vi "New Message.vi"(0 "Message Maker in":refnum<class "Message Maker.lvclass">, 5 "Method Qualified Name":string, 11 "error in (no error)":errorcluster, 12 "Message Type":T1) -> (3 "Message Recipient Type":T2, 4 "Message Maker out":refnum<class "Message Maker.lvclass">, 6 "References":T3, 8 "AF Library FQN":string, 10 "Async AF Library FQN":string, 14 "Updating?":bool, 15 "error out":errorcluster)   [LabVIEW 2023, in "Message Maker.lvclass"]
doc: "Sets up the method to be built. If this is a new message, it will copy over the template. If this is a message to be updated it resets the old message\n\nAuthor: Derek Trepanier\nCopyright: MGI 2015"
uses:
  Message Maker.lvclass
  Scripting Refs.ctl
  Message Recipient Type.ctl
  Message Type.ctl
  Message Maker.lvclass/Message Maker.ctl
  <vilib>/Utility/error.llb/Error Cluster From Error Code.vi
  <vilib>/ErrorRing/Error Ring.xnode
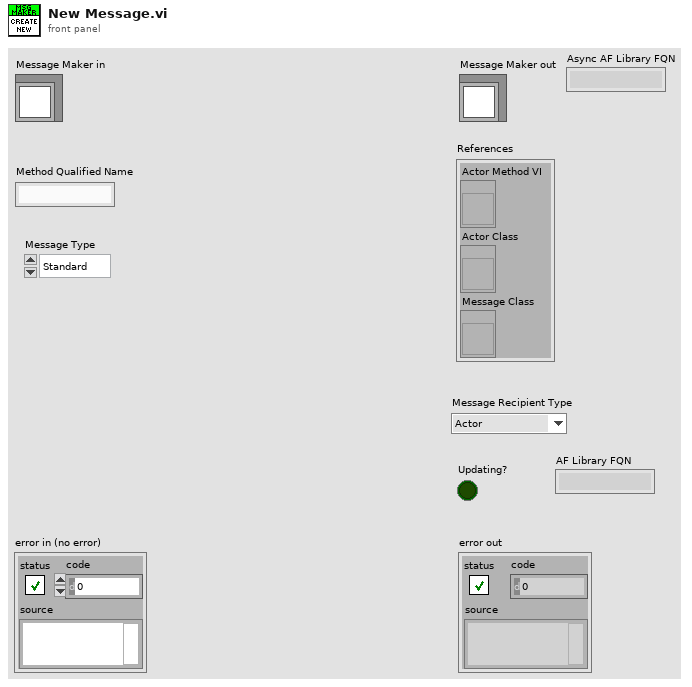
[diagram p1: front panel]
types:
  T1 = typedef "Message Maker.lvclass/Message Type.ctl" = enum16{"Standard", "Async"}
  T2 = typedef "Message Maker.lvclass/Message Recipient Type.ctl" = enum16{"Actor", "Interface", "Async Actor"}
  T3 = typedef "Message Maker.lvclass/Scripting Refs.ctl" = cluster{"Actor Method VI":refnum<vi>, "Actor Class":refnum<vi>, "Message Class":refnum<vi>}
  T4 = typedef "Message Maker.lvclass/Messages Map.ctl" = map{string, T5}
  T5 = typedef "Message Maker.lvclass/Message Details.ctl" = cluster{"Message Ref":refnum<vi>, "Message Type":T1}
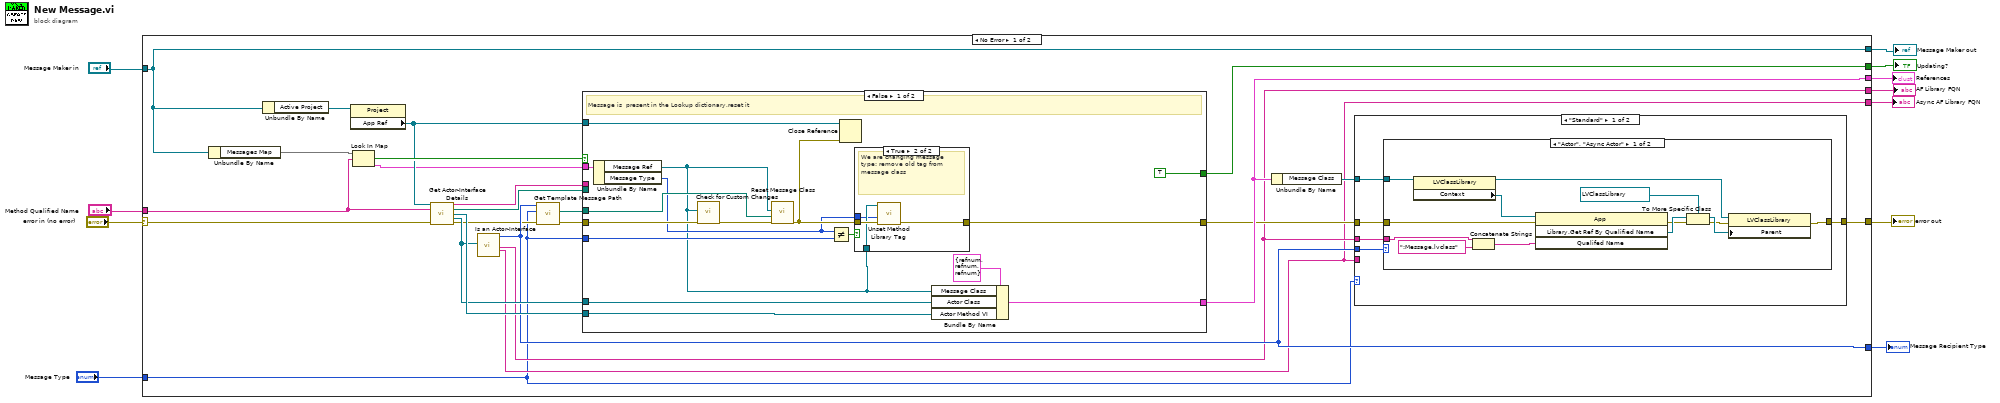
[diagram p0: block diagram]
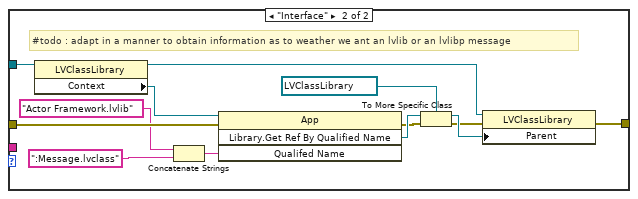
[diagram p2: hidden frame]
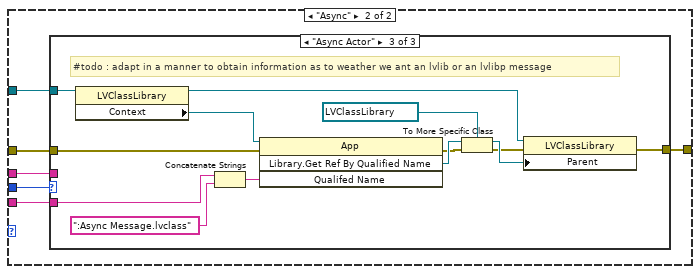
[diagram p3: hidden frame]
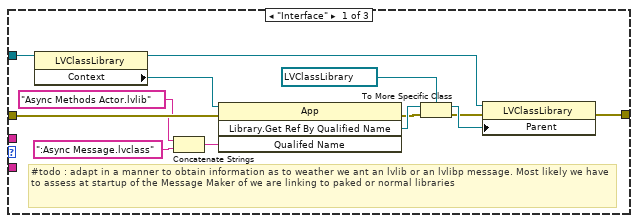
[diagram p4: hidden frame]
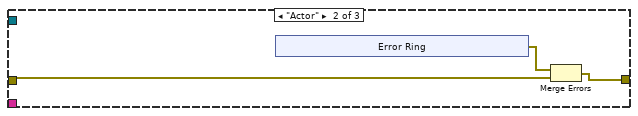
[diagram p5: hidden frame]
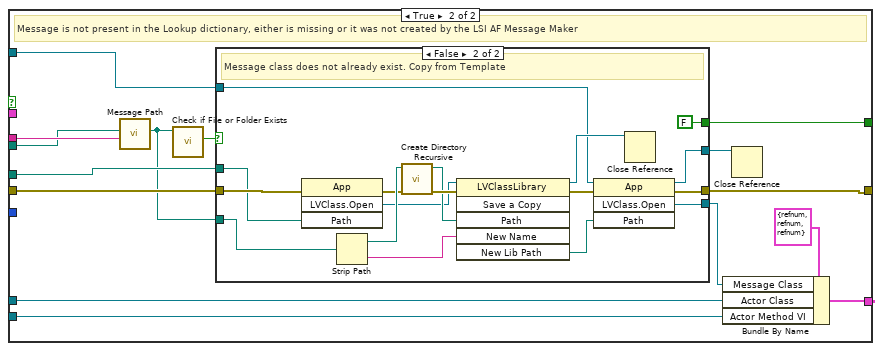
[diagram p7: hidden frame]
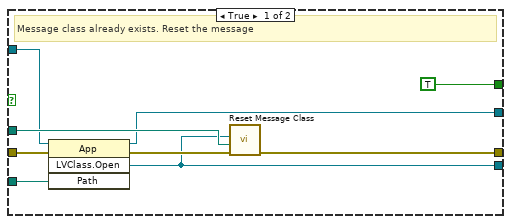
[diagram p8: hidden frame]
diagram:
  n1 = case shown="No Error" "error in (no error)" {
    selector: "error in (no error)" -> [w28 w169]
    tunnel: [w31 w169] -> w10
    tunnel: [w20 w168] -> w8
    tunnel: "Message Maker in" -> [w20 w168]
    tunnel: "Method Qualified Name" -> [w27 _]
    tunnel: [w33 _] -> w6
    tunnel: [w34 _] -> w5
    tunnel: [w15 _] -> w4
    tunnel: [w18 _] -> w3
    tunnel: "Message Type" -> [w12 _]
    tunnel: [w14 _] -> w1
    frame No Error {
      n2 = Unbundle By Name(w20) -> ("Messages Map"=w19:T4)
      n3 = Unbundle By Name(w20) -> ("Active Project"=w29:refnum<vi>)
      n4 = property class="Project"(reference=w29) -> ("App Ref"=w26:refnum<vi>)  [unwired: 1 in, 2 out]
      n5 = Look In Map(map=w19, key=w27) -> (key not found?=w35:bool, value=w13:T5)  [unwired: 1 in]
      n6 = call "Get Actor-Interface Details.vi"("Application"=w26, "Method Qualified Name"=w27, "error in (no error)"=w28) -> ("Actor Name"=w25:string, "Actor Path"=w24:path, "Actor Method VI Reference"=w23:refnum<vi>, "Actor Reference"=w21:refnum<vi>, "error out"=w17:errorcluster)  [unwired: 8 in]
      n7 = call "Is an Actor-Interface.vi"("Class in"=w21) -> ("Message Recipient Type"=w18:T2, "AF Library FQN"=w15:string, "Async AF Library FQN"=w14:string)  [unwired: 14 in, 2 out]
      n8 = call "Get Template Message Path.vi"("error in"=w17, "Message Type"=w12, "Message Recipient Type"=w18) -> ("error out"=w16:errorcluster, "appended path"=w22:path)  [unwired: 7 in]
      n9 = case shown="False" w35 {
        tunnel: [w119 w128] -> w33
        tunnel: w16 -> [w117 w139]
        tunnel: [w112 w129] -> w30
        tunnel: w22 -> [w121 w137]
        tunnel: [TRUE w136] -> w34
        tunnel: w26 -> [w115 w135]
        tunnel: w25 -> [_ w134]
        tunnel: w24 -> [_ w133]
        tunnel: w21 -> [w111 w132]
        tunnel: w23 -> [w114 w131]
        tunnel: w13 -> [w110 _]
        tunnel: w12 -> [w109 _]
        frame False {
          # "Message is  present in the Lookup dictionary,reset it"
          n10 = Unbundle By Name(w110) -> ("Message Ref"=w106:refnum<vi>, "Message Type"=w107:T1)
          n11 = call "Check for Custom Changes.vi"("error in (no error)"=w117, "Message Class"=w106) -> ("error out"=w116:errorcluster)  [unwired: 9 in]
          n12 = call "Reset Message Class.vi"("error in (no error)"=w116, "Template Path"=w121, "Message Class"=w106) -> ("error out"=w113:errorcluster)  [unwired: 8 in]
          n13 = Not Equal?(x=w107, y=w109) -> (x != y?=w108:bool)
          n14 = Close Reference(reference=w115, error in (no error)=w113) -> ()  [unwired: 1 out]
          n15 = case shown="True" w108 {
            tunnel: w113 -> [w122 w126]
            tunnel: [w122 w125] -> w112
            tunnel: w106 -> [_ w124]
            tunnel: w107 -> [_ w123]
            frame False {
            }
            frame True {
              # "We are changing message type: remove old tag from message class"
              n16 = call "Unset Method Library Tag.vi"("error in (no error)"=w126, "Message Type"=w123, "LVClassLibrary in"=w124) -> ("error out"=w125:errorcluster)  [unwired: 7 in, 1 out]
            }
          }
          n17 = Bundle By Name(cluster=T3 {"Actor Method VI"=refnum, "Actor Class"=refnum, "Message Class"=refnum} ("References"), "Message Class"=w106, "Actor Class"=w111, "Actor Method VI"=w114) -> (w119:T3)
        }
        frame True {
          # "Message is not present in the Lookup dictionary, either is missing or it was not created by the LSI AF Message Maker"
          n18 = call "Message Path.vi"("Message Method"=w134, "Class Path"=w133) -> ("Message Class Path"=w130:path)  [unwired: 9 in]
          n19 = call <vilib>:"Check if File or Folder Exists.vi"("path"=w130) -> ("file or folder exists?"=w127:bool)  [unwired: 8 in, 2 out]
          n20 = case shown="False" w127 {
            tunnel: w130 -> [w148 w161]
            tunnel: w139 -> [w145 w159]
            tunnel: w135 -> [w149 w158]
            tunnel: [w143 w155] -> w140
            tunnel: [w144 w154] -> w129
            tunnel: [w147 w153] -> w138
            tunnel: w137 -> [w150 w152]
            tunnel: [TRUE FALSE] -> w136
            frame True {
              # "Message class already exists. Reset the message"
              n21 = invoke class="App" method="LVClass.Open"(reference=w149, error in=w145, "Path"=w148) -> (reference out=w147:refnum<vi>, error out=w146:errorcluster, "LVClass.Open"=w143:refnum<vi>)  [unwired: 1 in, 1 out]
              n22 = call "Reset Message Class.vi"("error in (no error)"=w146, "Template Path"=w150, "Message Class"=w143) -> ("error out"=w144:errorcluster)  [unwired: 8 in]
            }
            frame False {
              # "Message class does not already exist. Copy from Template"
              n23 = invoke class="App" method="LVClass.Open"(error in=w159, "Path"=w152) -> (error out=w160:errorcluster, "LVClass.Open"=w163:refnum<vi>)  [unwired: 2 in, 2 out]
              n24 = Strip Path(path=w161) -> (stripped path=w165:path, name=w162:string)
              n25 = call <vilib>:"Create Directory Recursive.vi"("error in (no error)"=w160, "directory"=w165) -> ("error out"=w167:errorcluster, "directory copy"=w166:path)  [unwired: 3 in, 1 out]
              n26 = invoke class="LVClassLibrary" method="Save a Copy"(reference=w163, error in=w167, "Path"=w166, "New Name"=w162) -> (reference out=w164:refnum<vi>, error out=w156:errorcluster, "New Lib Path"=w157:path)  [unwired: 2 in, 3 out]
              n27 = invoke class="App" method="LVClass.Open"(reference=w158, error in=w156, "Path"=w157) -> (reference out=w153:refnum<vi>, error out=w154:errorcluster, "LVClass.Open"=w155:refnum<vi>)  [unwired: 1 in, 1 out]
              n28 = Close Reference(reference=w164) -> ()  [unwired: 1 in, 1 out]
            }
          }
          n29 = Bundle By Name(cluster=T3 {"Actor Method VI"=refnum, "Actor Class"=refnum, "Message Class"=refnum} ("References"), "Message Class"=w140, "Actor Class"=w132, "Actor Method VI"=w131) -> (w128:T3)
          n30 = Close Reference(reference=w138) -> ()  [unwired: 1 in, 1 out]
        }
      }
      n31 = Unbundle By Name(w33) -> ("Message Class"=w32:refnum<vi>)
      n32 = case shown="\"Standard\"" w12 {
        tunnel: w32 -> [w40 w72]
        tunnel: [w39 w71] -> w31
        tunnel: w30 -> [w38 w70]
        tunnel: w15 -> [w37 w69]
        tunnel: w18 -> [w36 w68]
        tunnel: w14 -> [_ w67]
        frame "Standard" {
          n33 = case shown="\"Actor\", \"Async Actor\"" w36 {
            tunnel: w40 -> [w53 w66]
            tunnel: [w52 w65] -> w39
            tunnel: w38 -> [w51 w64]
            tunnel: w37 -> [w41 _]
            frame "Actor", "Async Actor" {
              n34 = property class="LVClassLibrary"(reference=w53) -> (reference out=w50:refnum<vi>, "Context"=w49:refnum<vi>)  [unwired: 1 in, 1 out]
              n35 = Concatenate Strings(w41, ":Message.lvclass" ("string")) -> (w42:string)
              n36 = invoke class="App" method="Library.Get Ref By Qualified Name"(reference=w49, error in=w51, "Qualifed Name"=w42) -> (error out=w45:errorcluster, "Library.Get Ref By Qualified Name"=w48:refnum<vi>)  [unwired: 1 in, 2 out]
              n37 = To More Specific Class(target class=refnum<vi> refnum ("Parent Class"), reference=w48, error in=w45) -> (specific class reference=w46:refnum<vi>, error out=w44:errorcluster)
              n38 = property class="LVClassLibrary"(reference=w50, error in=w44, "Parent"=w46) -> (error out=w52:errorcluster)  [unwired: 1 out]
            }
            frame "Interface" {
              # "#todo : adapt in a manner to obtain information as to weather we ant an lvlib or an lvlibp message"
              n39 = property class="LVClassLibrary"(reference=w66) -> (reference out=w63:refnum<vi>, "Context"=w62:refnum<vi>)  [unwired: 1 in, 1 out]
              n40 = Concatenate Strings("Actor Framework.lvlib" ("Actor Class"), ":Message.lvclass" ("string")) -> (w55:string)
              n41 = invoke class="App" method="Library.Get Ref By Qualified Name"(reference=w62, error in=w64, "Qualifed Name"=w55) -> (error out=w58:errorcluster, "Library.Get Ref By Qualified Name"=w61:refnum<vi>)  [unwired: 1 in, 2 out]
              n42 = To More Specific Class(target class=refnum<vi> refnum ("Parent Class"), reference=w61, error in=w58) -> (specific class reference=w59:refnum<vi>, error out=w57:errorcluster)
              n43 = property class="LVClassLibrary"(reference=w63, error in=w57, "Parent"=w59) -> (error out=w65:errorcluster)  [unwired: 1 out]
            }
          }
        }
        frame "Async" {
          n44 = case shown="\"Async Actor\"" w68 {
            tunnel: w72 -> [w85 _ w105]
            tunnel: [w84 w86 w104] -> w71
            tunnel: w70 -> [w83 w87 w103]
            tunnel: w69 -> [_ _ _]
            tunnel: w67 -> [_ _ w93]
            frame "Interface" {
              # "#todo : adapt in a manner to obtain information as to weather we ant an lvlib or an lvlibp message. Most likely we have to assess at startup of the Message Maker of we are linking to paked or normal libraries"
              n45 = property class="LVClassLibrary"(reference=w85) -> (reference out=w82:refnum<vi>, "Context"=w81:refnum<vi>)  [unwired: 1 in, 1 out]
              n46 = Concatenate Strings("Async Methods Actor.lvlib" ("Actor Class"), ":Async Message.lvclass" ("string")) -> (w74:string)
              n47 = invoke class="App" method="Library.Get Ref By Qualified Name"(reference=w81, error in=w83, "Qualifed Name"=w74) -> (error out=w77:errorcluster, "Library.Get Ref By Qualified Name"=w80:refnum<vi>)  [unwired: 1 in, 2 out]
              n48 = To More Specific Class(target class=refnum<vi> refnum ("Parent Class"), reference=w80, error in=w77) -> (specific class reference=w78:refnum<vi>, error out=w76:errorcluster)
              n49 = property class="LVClassLibrary"(reference=w82, error in=w76, "Parent"=w78) -> (error out=w84:errorcluster)  [unwired: 1 out]
            }
            frame "Actor" {
              n50 = xnode "Error Ring"() -> ("error out"=w88:errorcluster)
              n51 = Merge Errors(w88, w87) -> (w86:errorcluster)
            }
            frame "Async Actor" {
              # "#todo : adapt in a manner to obtain information as to weather we ant an lvlib or an lvlibp message"
              n52 = property class="LVClassLibrary"(reference=w105) -> (reference out=w102:refnum<vi>, "Context"=w101:refnum<vi>)  [unwired: 1 in, 1 out]
              n53 = Concatenate Strings(w93, ":Async Message.lvclass" ("string")) -> (w95:string)
              n54 = invoke class="App" method="Library.Get Ref By Qualified Name"(reference=w101, error in=w103, "Qualifed Name"=w95) -> (error out=w97:errorcluster, "Library.Get Ref By Qualified Name"=w100:refnum<vi>)  [unwired: 1 in, 2 out]
              n55 = To More Specific Class(target class=refnum<vi> refnum ("Parent Class"), reference=w100, error in=w97) -> (specific class reference=w98:refnum<vi>, error out=w96:errorcluster)
              n56 = property class="LVClassLibrary"(reference=w102, error in=w96, "Parent"=w98) -> (error out=w104:errorcluster)  [unwired: 1 out]
            }
          }
        }
      }
    }
    frame Error {
    }
  }
  "error out" <- w10
  "Message Maker out" <- w8
  "References" <- w6
  "Updating?" <- w5
  "AF Library FQN" <- w4
  "Message Recipient Type" <- w3
  "Async AF Library FQN" <- w1
